vi "VIH - CHM Project - Read HHP File.vi"(8 "error in":errorcluster, 11 "HHP File":path) -> (0 "error out":errorcluster, 2 "Files":T1, 3 "dup HHP File":path)   [LabVIEW 2014]
doc: "::: VI Helpeks :::\nCopyright (c) 2000-2026 Konstantin Shifershteyn. All rights reserved."
panel:
  # "VI Helpeks\nCopyright (c) 2012-2026 Konstantin Shifershteyn"
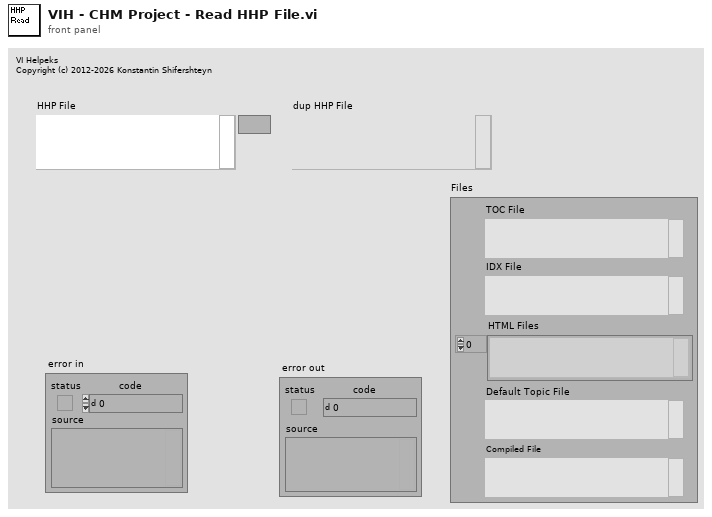
[diagram p1: front panel]
types:
  T1 = cluster{"TOC File":path, "IDX File":path, "HTML Files":path[], "Default Topic File":path, "Compiled File":path}
  T2 = typedef "VIH - CHM Project - HHP Support - Queue Refnum.ctl" = refnum<queue>
  T3 = cluster{"Path out":path, "Path out":path, path[], "Path out":path, "Path out":path}
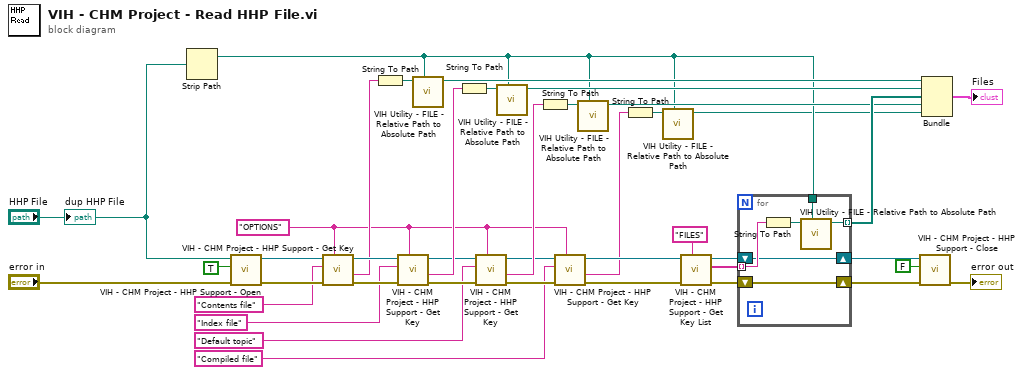
[diagram p0: block diagram]
diagram:
  w8 = "OPTIONS" ("Section")
  n1 = Strip Path(path="HHP File") -> (stripped path=w2:path)  [unwired: 1 out]
  n2 = call "VIH - CHM Project - HHP Support - Open.vi"("error in"="error in", "must exist (F)"=TRUE, "Config File"="HHP File") -> ("error out"=w36:errorcluster, "queue out"=w37:T2)  [unwired: 7 in]
  n3 = call "VIH - CHM Project - HHP Support - Get Key.vi"("Section"=w8, "error in"=w36, "Key"="Contents file", "queue"=w37) -> ("error out"=w33:errorcluster, "Value"=w25:string, "dup queue"=w34:T2)  [unwired: 4 in, 1 out]
  n4 = String To Path(string=w25) -> (path=w24:path)
  n5 = call "VIH - CHM Project - HHP Support - Get Key.vi"("Section"=w8, "error in"=w33, "Key"="Index file", "queue"=w34) -> ("error out"=w16:errorcluster, "Value"=w22:string, "dup queue"=w17:T2)  [unwired: 4 in, 1 out]
  n6 = call "VIH Utility - FILE - Relative Path to Absolute Path.vi"("base path (empty: dir of Top VI)"=w2, "Path"=w24) -> ("Path out"=w20:path)  [unwired: 8 in, 1 out]
  n7 = String To Path(string=w22) -> (path=w23:path)
  n8 = call "VIH - CHM Project - HHP Support - Get Key.vi"("Section"=w8, "error in"=w16, "Key"="Default topic", "queue"=w17) -> ("error out"=w9:errorcluster, "Value"=w13:string, "dup queue"=w10:T2)  [unwired: 4 in, 1 out]
  n9 = call "VIH Utility - FILE - Relative Path to Absolute Path.vi"("base path (empty: dir of Top VI)"=w2, "Path"=w23) -> ("Path out"=w19:path)  [unwired: 8 in, 1 out]
  n10 = String To Path(string=w13) -> (path=w14:path)
  n11 = call "VIH - CHM Project - HHP Support - Get Key.vi"("Section"=w8, "error in"=w9, "Key"="Compiled file", "queue"=w10) -> ("error out"=w6:errorcluster, "Value"=w3:string, "dup queue"=w7:T2)  [unwired: 4 in, 1 out]
  n12 = call "VIH Utility - FILE - Relative Path to Absolute Path.vi"("base path (empty: dir of Top VI)"=w2, "Path"=w14) -> ("Path out"=w11:path)  [unwired: 8 in, 1 out]
  n13 = String To Path(string=w3) -> (path=w4:path)
  n14 = call "VIH Utility - FILE - Relative Path to Absolute Path.vi"("base path (empty: dir of Top VI)"=w2, "Path"=w4) -> ("Path out"=w1:path)  [unwired: 8 in, 1 out]
  n15 = call "VIH - CHM Project - HHP Support - Get Key List.vi"("Section"="FILES", "error in"=w6, "queue"=w7) -> ("error out"=w30:errorcluster, "Keys"=w29:string[], "dup queue"=w31:T2)  [unwired: 6 in]
  n16 = for {
    tunnel: w29 -> [w44] mode=indexing
    shift-right: [w43] -> w26
    shift-left: w31 -> [w43]
    shift-right: [w42] -> w27
    shift-left: w30 -> [w42]
    tunnel: w2 -> [w46]
    tunnel: [w45] -> w12 mode=indexing
    n17 = String To Path(string=w44) -> (path=w47:path)
    n18 = call "VIH Utility - FILE - Relative Path to Absolute Path.vi"("base path (empty: dir of Top VI)"=w46, "Path"=w47) -> ("Path out"=w45:path)  [unwired: 8 in, 1 out]
  }
  n19 = call "VIH - CHM Project - HHP Support - Close.vi"("error in"=w27, "write file (F)"=FALSE, "queue"=w26) -> ("error out"=→"error out":errorcluster)  [unwired: 8 in]
  n20 = Bundle("Path out"=w20, "Path out"=w19, w12, "Path out"=w11, "Path out"=w1) -> (→"Files":T3)  [unwired: 1 in]
  "dup HHP File" <- "HHP File"
